vi "RegisterImagePtr.vi"(8 "error in":errorcluster, 11 "Image Reference In":T3) -> (0 "error out":errorcluster, 2 "ImagePointer":T1 {"ImagePointer" format="%.0x"}, 3 "Image Reference Out":T3)   [LabVIEW 2020, in "OpenLvVision_Image.lvlib" / "DataAccess.lvlib"]
doc: "Provides the image's memory pointer and alignment details."
uses:
  DataAccess.lvlib
  Management/TypeDef/Image.ctl
  TypeDef/ImagePointer.ctl
  Management/TypeDef/ImageType.ctl
  Management/Management.lvlib
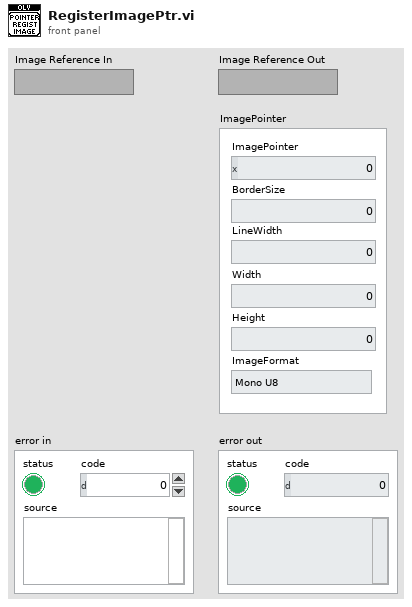
[diagram p1: front panel]
types:
  T1 = typedef "OpenLvVision_Image.lvlib/DataAccess.lvlib/ImagePointer.ctl" = cluster{"ImagePointer":u64, "BorderSize":i32, "LineWidth":i32, "Width":i32, "Height":i32, "ImageFormat":T2}
  T2 = typedef "OpenLvVision_Image.lvlib/Management.lvlib/ImageType.ctl" = enum16{"Mono U8", "Mono U16", "Mono I16", "Mono SGL", "Color U32", "Color U64"}
  T3 = typedef "OpenLvVision_Image.lvlib/Management.lvlib/Image.ctl" = refnum<image>
  T4 = typedef "OpenLvVision_Image.lvlib/DataAccess.lvlib/PixelPointer.ctl" = cluster{"Image Border Size":i32, "Pixel Pointer":u64, "LineWidth":i32, "PixelSize_Bytes":i32, "TransferMaxSize":i32}
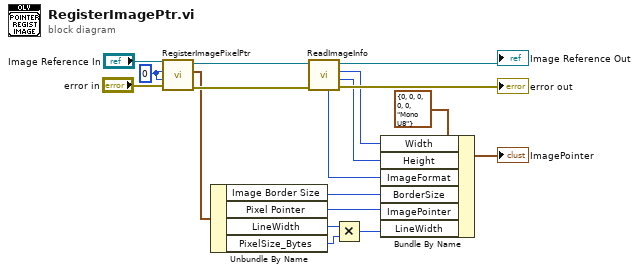
[diagram p0: block diagram]
diagram:
  w1 = 0
  n1 = call "RegisterImagePixelPtr.vi"("error in"="error in", "Y Coordinate"=w1, "X Coordinate"=w1, "Image Reference In"="Image Reference In") -> ("error out"=w15:errorcluster, "PixelPointer"=w7:T4, "Image Reference Out"=w16:T3)  [unwired: 5 in]
  n2 = Unbundle By Name(w7) -> ("Image Border Size"=w6:i32, "Pixel Pointer"=w5:u64, "LineWidth"=w4:i32, "PixelSize_Bytes"=w3:i32)
  n3 = call "ReadImageInfo.vi"("error in"=w15, "Image Reference In"=w16) -> ("error out"=→"error out":errorcluster, "Height"=w9:i32, "Width"=w10:i32, "Image Reference Out"=→"Image Reference Out":T3, "Image Type"=w8:T2)  [unwired: 4 in, 1 out]
  n4 = Multiply(x=w4, y=w3) -> (x*y=w2:i32)
  n5 = Bundle By Name(cluster=T1 {"ImagePointer"=0, "BorderSize"=0, "LineWidth"=0, "Width"=0, "Height"=0, "ImageFormat"=enum."Mono U8"} ("ImagePointer"), "Width"=w10, "Height"=w9, "ImageFormat"=w8, "BorderSize"=w6, "ImagePointer"=w5, "LineWidth"=w2) -> (→"ImagePointer":T1)
